vi "contains_item.vi"(8 "error in (no error)":errorcluster, 10 "item_name":string, 11 "Table in":refnum<class "Table.lvclass">) -> (0 "error out":errorcluster, 2 "contains_item":bool, 3 "Table out":refnum<class "Table.lvclass">)   [LabVIEW 2020, in "toml_edit.lvlib" / "Table.lvclass"]
uses:
  Table.lvclass
  Table.lvclass/Table.ctl
  dragon_toml_64.dll
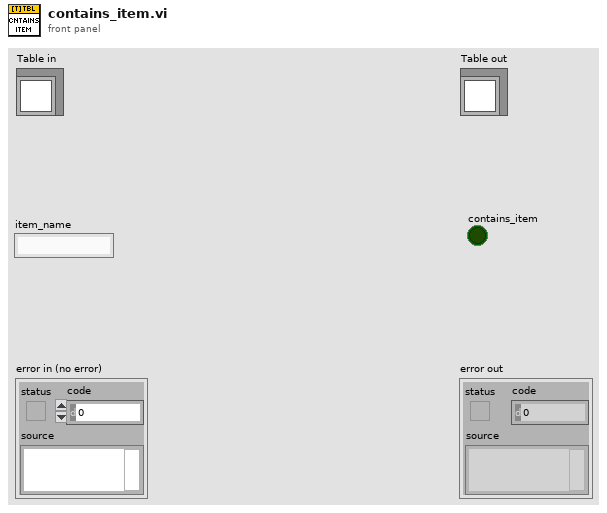
[diagram p1: front panel]
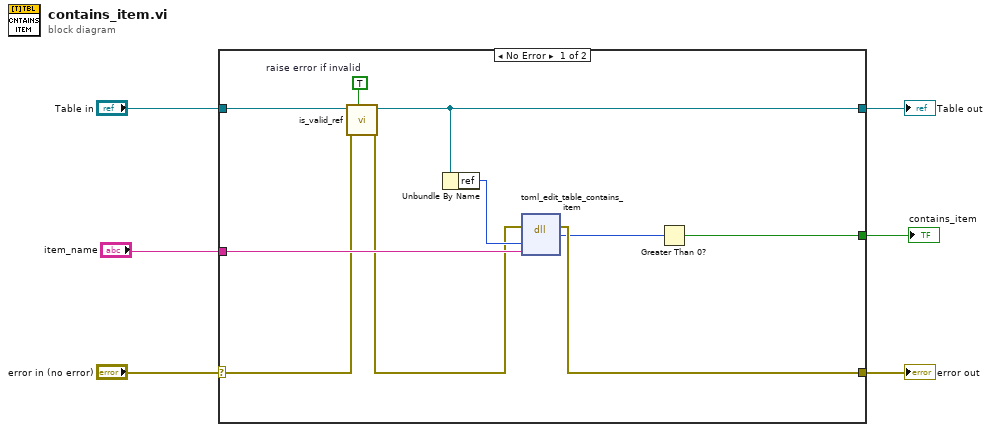
[diagram p0: block diagram]
diagram:
  n1 = case shown="No Error" "error in (no error)" {
    selector: "error in (no error)" -> [w8 w18]
    tunnel: [w14 w18] -> w5
    tunnel: [w9 w17] -> w3
    tunnel: "Table in" -> [w10 w17]
    tunnel: "item_name" -> [w15 _]
    tunnel: [w12 _] -> w1
    frame No Error {
      w11 = TRUE  # raise error if invalid
      n2 = call-dynamic "is_valid_ref.vi"("raise error if invalid? (False)"=w11, "error in (no error)"=w8, "Table in"=w10) -> ("error out"=w7:errorcluster, "Table out"=w9:refnum<class "Table.lvclass">)  [unwired: 6 in, 1 out]
      n3 = Unbundle By Name(w9) -> ("ref"=w16:u64)
      n4 = dll-call lib="C:/projects/dragon-desktop/source/submodules/toml-edit-labview/lv_src/dragon_toml_*.*" fn="toml_edit_table_contains_item"(error in=w7, "table_ref"=w16, "item_name"=w15) -> (error out=w14:errorcluster, "contains_item_bool"=w13:u64)  [unwired: 4 in, 1 out]
      n5 = Greater Than 0?(x=w13) -> (x > 0?=w12:bool)
    }
    frame Error {
    }
  }
  "error out" <- w5
  "Table out" <- w3
  "contains_item" <- w1
